vi "Get Tx Scheduled Label Configuration.vi"(8 "error in":errorcluster, 10 "configuration string":string, 11 "port":T1 format="%.0x") -> (0 "error out":errorcluster, 2 "configuration string out":string, 3 "port out":T1 format="%.0x")   [LabVIEW 2020, in "Ballard ARINC 429 Hardware Configuration.lvlib"]
uses:
  Ballard ARINC 429 Hardware Configuration.lvlib
  <vilib>/NI VeriStand/Custom Device API/Custom Device Item Ref.ctl
  Constants.vi
  Scripting/Ballard/Ballard ARINC 429 Scripting.lvlib
  Scripting/ARINC 429/ARINC 429 Scripting.lvlib
  <vilib>/NI VeriStand/Custom Device API/Custom Device API.lvlib
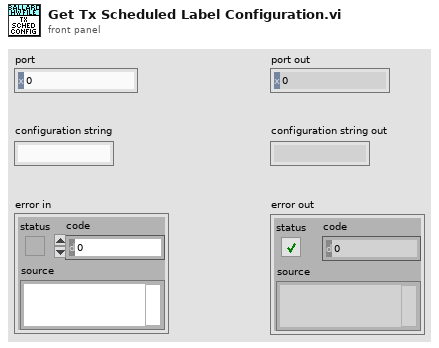
[diagram p1: front panel]
types:
  T1 = typedef "Custom Device API.lvlib/Custom Device Item Ref.ctl" = u64
  T2 = typedef "Label Properties.ctl" = cluster{"label (Dec)":T3, "SDI value":u8, "SDI enabled":bool}
  T3 = typedef "Label.ctl" = u8
  T4 = typedef "Transfer Type.ctl" = enum16{"Scheduled", "Acyclic", "Block", "Strobe"}
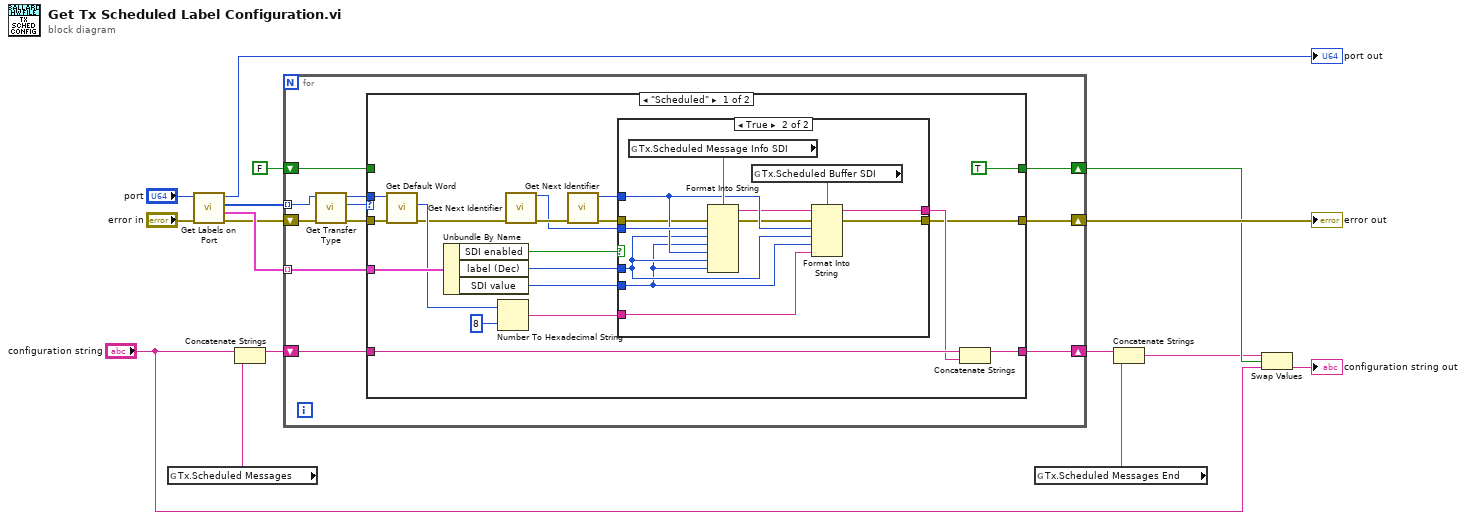
[diagram p0: block diagram]
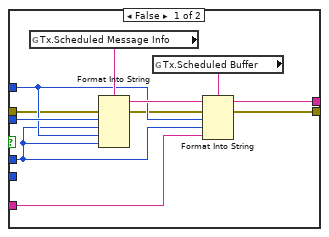
[diagram p2: hidden frame]
diagram:
  n1 = global read "Constants.vi" "Tx.Scheduled Messages"() -> (w2:string)
  n2 = call "Get Labels on Port.vi"("error in"="error in", "port in"="port") -> ("error out"=w10:errorcluster, "labels properties"=w12:T2[], "labels"=w11:T1[], "port out"=→"port out":T1)  [unwired: 6 in]
  n3 = Concatenate Strings("configuration string", w2) -> (w13:string)
  n4 = for {
    shift-right: [w25] -> w8
    shift-left: w13 -> [w26]
    tunnel: w12 -> [w27] mode=indexing
    tunnel: w11 -> [w23] mode=indexing
    shift-right: [w24] -> w9
    shift-left: w10 -> [w18]
    shift-right: [w19] -> w6
    shift-left: FALSE -> [w20]
    n5 = call "Get Transfer Type.vi"("error in"=w18, "label ref in"=w23) -> ("error out"=w17:errorcluster, "transfer type"=w21:T4, "label ref out"=w22:T1)  [unwired: 7 in]
    n6 = case shown="\"Scheduled\"" w21 {
      tunnel: w27 -> [w46 _]
      tunnel: w17 -> [w38 w72]
      tunnel: w26 -> [w42 w71]
      tunnel: [w41 w71] -> w25
      tunnel: [w29 w72] -> w24
      tunnel: w22 -> [w40 _]
      tunnel: w20 -> [_ w70]
      tunnel: [TRUE w70] -> w19
      frame "Scheduled" {
        n7 = call "Get Default Word.vi"("error in"=w38, "Item Ref in"=w40) -> ("error out"=w37:errorcluster, "default word"=w44:u32)  [unwired: 7 in, 1 out]
        n8 = Unbundle By Name(w46) -> ("SDI enabled"=w33:bool, "label (Dec)"=w32:T3, "SDI value"=w35:u8)
        n9 = Number To Hexadecimal String(1:i16 8 ("width (-)"), 2:w44) -> (0:w28:string)
        n10 = call "Get Next Identifier.vi"("error in"=w37) -> ("error out"=w45:errorcluster, "ID"=w36:u32)  [unwired: 9 in]
        n11 = call "Get Next Identifier.vi"("error in"=w45) -> ("error out"=w30:errorcluster, "ID"=w34:u32)  [unwired: 9 in]
        n12 = case shown="True" w33 {
          tunnel: [w54 w65] -> w31
          tunnel: w36 -> [w56 w68]
          tunnel: w35 -> [_ w59]
          tunnel: w34 -> [w52 w66]
          tunnel: w32 -> [w48 w60]
          tunnel: w30 -> [w51 w63]
          tunnel: [w49 w61] -> w29
          tunnel: w28 -> [w47 w58]
          frame False {
            n13 = global read "Constants.vi" "Tx.Scheduled Message Info"() -> (w57:string)
            n14 = Format Into String(format string=w57, error in=w51, w56, w48, w52, w48) -> (resulting string=w55:string, error out=w50:errorcluster)  [unwired: 1 in]
            n15 = global read "Constants.vi" "Tx.Scheduled Buffer"() -> (w53:string)
            n16 = Format Into String(format string=w53, initial string=w55, error in=w50, w52, w48, w47) -> (resulting string=w54:string, error out=w49:errorcluster)
          }
          frame True {
            n17 = global read "Constants.vi" "Tx.Scheduled Message Info SDI"() -> (w69:string)
            n18 = Format Into String(format string=w69, error in=w63, w68, w60, w59, w66, w60, w59) -> (resulting string=w64:string, error out=w62:errorcluster)  [unwired: 1 in]
            n19 = global read "Constants.vi" "Tx.Scheduled Buffer SDI"() -> (w67:string)
            n20 = Format Into String(format string=w67, initial string=w64, error in=w62, w66, w60, w59, w58) -> (resulting string=w65:string, error out=w61:errorcluster)
          }
        }
        n21 = Concatenate Strings(w42, w31) -> (w41:string)
      }
      frame Default {
      }
    }
  }
  "error out" <- w9
  n22 = global read "Constants.vi" "Tx.Scheduled Messages End"() -> (w1:string)
  n23 = Concatenate Strings(w8, w1) -> (w5:string)
  n24 = Swap Values(12:w5, 13:w6, 14:"configuration string") -> (3:→"configuration string out":string)  [unwired: 1 out]
